vi "F1_Save_Array.vi"(9 "File Path":path, 10 "Format":string, 11 "Data":dbl[][](array[numeric])) -> (2 "error out":errorcluster, 3 "spreadsheet string":string)   [LabVIEW 2026]
doc: "Use this template to build a VI to use as a subVI."
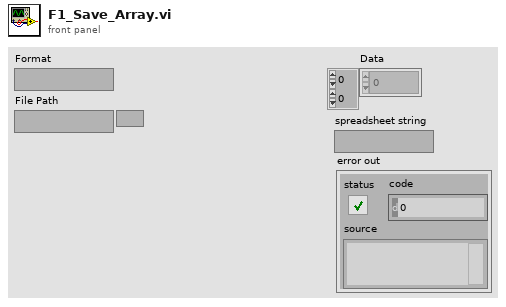
[diagram p1: front panel]
types:
  T1 = enum16{"open", "replace", "create", "open or create", "replace or create", "replace or create with confirmation"}
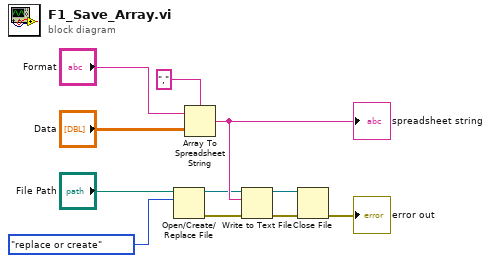
[diagram p0: block diagram]
diagram:
  n1 = Open/Create/Replace File(file path (use dialog)="File Path", operation (0:open)=T1."replace or create") -> (refnum out=w5:refnum<file>, error out=w4:errorcluster)  [unwired: 4 in, 1 out]
  n2 = Array To Spreadsheet String(delimiter (Tab)=",", array="Data", 3:"Format") -> (spreadsheet string=w8:string)
  "spreadsheet string" <- w8
  n3 = Write to Text File(file (use dialog)=w5, text=w8, error in=w4) -> (refnum out=w3:refnum<file>, error out=w2:errorcluster)  [unwired: 1 in, 1 out]
  n4 = Close File(refnum=w3, error in=w2) -> (error out=→"error out":errorcluster)  [unwired: 1 out]
